vi "AIO-DAQ-Panel.vi"(7 "Set(F)":bool, 8 "error in (no error)":errorcluster, 10 "First Time(F)":bool, 11 "object in":refnum<class>) -> (0 "error out":errorcluster, 2 "Changed?":bool, 3 "object out":refnum<class>)   [LabVIEW 2021, in "DAQmx.lvlib" / "AIO-Configuration.lvclass"]
uses:
  AIO-Configuration.lvclass
  Dependencies/AIO-Channel.lvlibp/AIO-Configuration_class/tdef/Direction.ctl
  C:/Users/averna/Documents/LV Gym DEMO/Factory Pattern/Device Channels/Dependencies/AIO-Channel.lvlibp/Channels/AIO-Channel/AIO-Configuration_class/AIO-Configuration.lvclass
  tdef/Data.ctl
  AIO-Configuration.lvclass/AIO-Configuration.ctl
  <resource>/objmgr/daqmx.rc
  DAQmx.lvlib
  C:/Users/averna/Documents/LV Gym DEMO/Factory Pattern/Device Channels/Dependencies/AIO-Channel.lvlibp/AIO-Configuration_class/AIO-Configuration.lvclass
  C:/Users/averna/Documents/LV Gym DEMO/Factory Pattern/Device Channels/Dependencies/Channel.lvlibp/Channel/Configuration_class/Configuration.lvclass
  C:/Users/averna/Documents/LV Gym DEMO/Factory Pattern/Device Channels/DAQmx/AIO-Configuration_class/AIO-Configuration.lvclass
  Dependencies/AIO-Channel.lvlibp/AIO-Configuration_class/AIO-Configuration.lvclass
panel:
  in  "Units":string
  in  "Scale":string(combo)
  in  "input terminal configuration":i32(ring)=-1 items=["Default"=-1, "RSE"=10083, "NRSE"=10078, "Differential"=10106, "Pseudodifferential"=12529]
  in  "minimum value":dbl=-5.0 format="%0.2f"
  in  "maximum value":dbl=5.0 format="%0.2f"
  in  "Direction":T1
  in  "Line":string(combo)
  in  "Device":string(combo)
  out "Not Saved?":bool
  in  "Save":bool
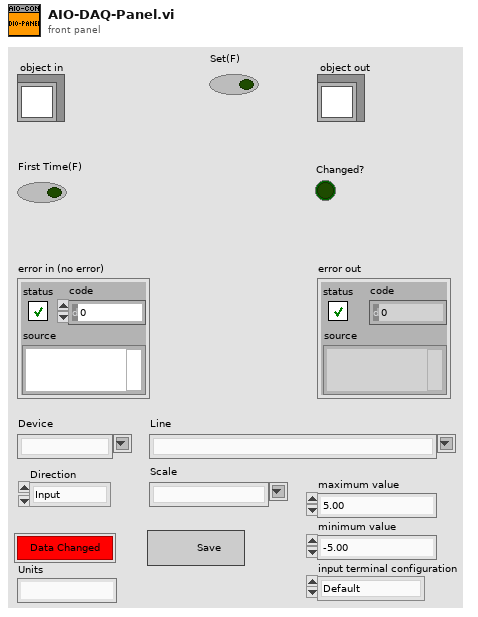
[diagram p1: front panel]
types:
  T1 = typedef "AIO-Channel.lvlibp/AIO-Configuration.lvclass/Direction.ctl" = enum16{"Input", "Output"}
  T2 = typedef "DAQmx.lvlib/AIO-Configuration.lvclass/Data.ctl" = cluster{"DAQ_Line":string, "maximum value":dbl, "minimum value":dbl, "input terminal configuration":i32, "custom scale name":string}
  T3 = cluster{"DAQ_Line":bool, "maximum value":bool, "minimum value":bool, "input terminal configuration":bool, "custom scale name":bool}
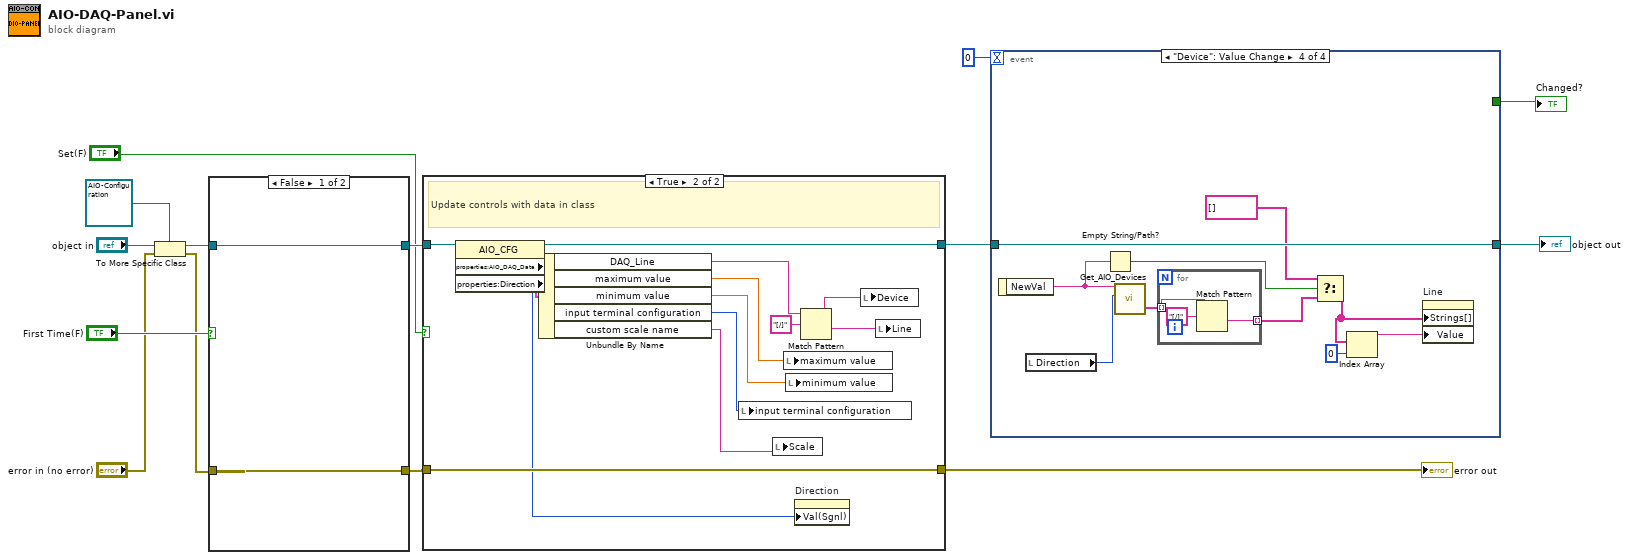
[diagram p0: block diagram]
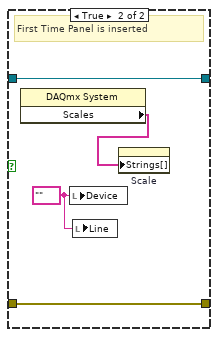
[diagram p2: hidden frame]
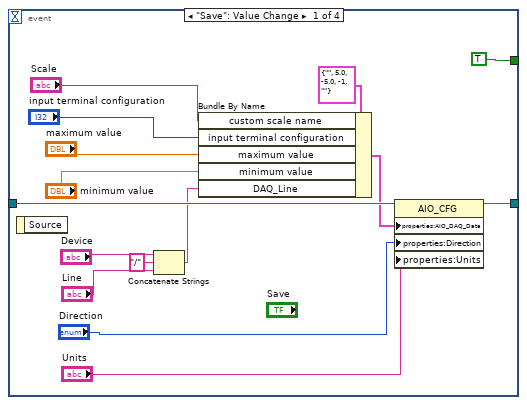
[diagram p3: hidden frame]
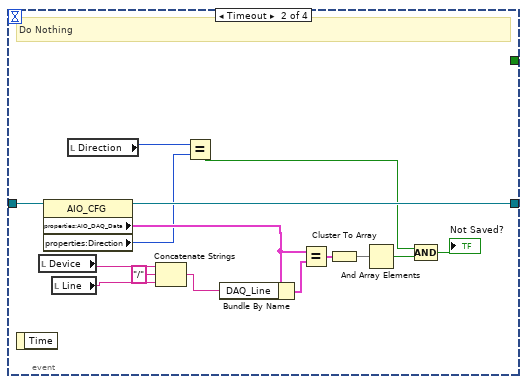
[diagram p4: hidden frame]
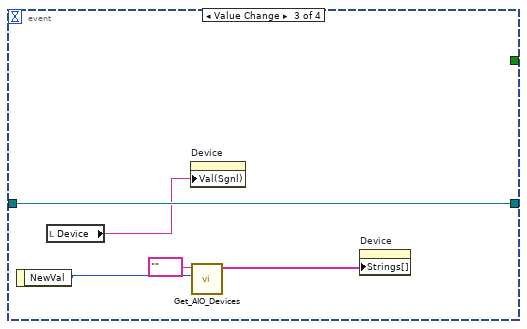
[diagram p5: hidden frame]
diagram:
  n1 = To More Specific Class(target class=refnum<class "AIO-Configuration.lvclass"> refnum ("Template-Channels.lvlib:Template_CFG"), reference="object in", error in="error in (no error)") -> (specific class reference=w8:refnum<class "AIO-Configuration.lvclass">, error out=w6:errorcluster)
  n2 = case shown="False" "First Time(F)" {
    tunnel: [w16 w20] -> w12
    tunnel: w8 -> [w16 w20]
    tunnel: [w15 w19] -> w11
    tunnel: w6 -> [w15 w19]
    frame False {
    }
    frame True {
      w18 = "" ("Device")
      # "First Time Panel is inserted"
      n3 = property class="DAQmx System"() -> ("Scales"=w17:tag[])  [unwired: 2 in, 2 out]
      n4 = local write "Device"(w18) -> ()
      n5 = local write "Line"(w18) -> ()
      n6 = property on="Scale" class="CmbBox"("Strings[]"=w17) -> ()  [unwired: 2 in, 2 out]
    }
  }
  n7 = case shown="True" "Set(F)" {
    tunnel: [w22 w33] -> w3
    tunnel: w12 -> [w22 w35]
    tunnel: [w21 w34] -> w10
    tunnel: w11 -> [w21 w34]
    frame False {
    }
    frame True {
      # "Update controls with data in class"
      n8 = property class="AIO_CFG"(reference=w35) -> (reference out=w33:refnum<class "AIO-Configuration.lvclass">, "properties:AIO_DAQ_Data"=w32:T2, "properties:Direction"=w27:T1)  [unwired: 1 in, 1 out]
      n9 = Unbundle By Name(w32) -> ("DAQ_Line"=w31:string, "maximum value"=w25:dbl, "minimum value"=w24:dbl, "input terminal configuration"=w26:i32, "custom scale name"=w23:string)
      n10 = local write "input terminal configuration"(w26) -> ()
      n11 = local write "Scale"(w23) -> ()
      n12 = local write "maximum value"(w25) -> ()
      n13 = local write "minimum value"(w24) -> ()
      n14 = property on="Direction" class="Enum (strict)"("Val(Sgnl)"=w27) -> ()  [unwired: 2 in, 2 out]
      n15 = Match Pattern(string=w31, regular expression="[/]") -> (before substring=w29:string, after substring=w28:string)  [unwired: 1 in, 2 out]
      n16 = local write "Device"(w29) -> ()
      n17 = local write "Line"(w28) -> ()
    }
  }
  "error out" <- w10
  n18 = event shown="[3] \"Device\": Value Change" {
    selector: _ -> [_ _ _ _]
    dyn-events: _ -> [_ _ _ _]
    timeout: 0 -> [_ _ _ _]
    tunnel: [w50 w64 w70 w80] -> w4
    tunnel: w3 -> [w49 w65 w70 w80]
    tunnel: [TRUE ("Changed?") _ _ _] -> w1
    event "Save": Value Change {
      n19 = event-data() -> ()  [unwired: 1 in, 1 out]
      n20 = Concatenate Strings("Device", "/" ("string"), "Line") -> (w37:string)
      n21 = Bundle By Name(cluster=T2 {"DAQ_Line"="", "maximum value"=5.0, "minimum value"=-5.0, "input terminal configuration"=-1, "custom scale name"=""} ("AIO_DAQ_Data"), "custom scale name"="Scale", "input terminal configuration"="input terminal configuration", "maximum value"="maximum value", "minimum value"="minimum value", "DAQ_Line"=w37) -> (w42:T2)
      n22 = property class="AIO_CFG"(reference=w49, "properties:AIO_DAQ_Data"=w42, "properties:Direction"="Direction", "properties:Units"="Units") -> (reference out=w50:refnum<class "AIO-Configuration.lvclass">)  [unwired: 1 in, 1 out]
    }
    event Timeout {
      # "Do Nothing"
      n23 = event-data() -> ()  [unwired: 1 in, 1 out]
      n24 = local read "Device"() -> (w58:string)
      n25 = property class="AIO_CFG"(reference=w65) -> (reference out=w64:refnum<class "AIO-Configuration.lvclass">, "properties:AIO_DAQ_Data"=w60:T2, "properties:Direction"=w53:T1)  [unwired: 1 in, 1 out]
      n26 = local read "Line"() -> (w57:string)
      n27 = local read "Direction"() -> (w54:T1)
      n28 = Concatenate Strings(w58, "/" ("string"), w57) -> (w55:string)
      n29 = Equal?(x=w54, y=w53) -> (x = y?=w51:bool)
      n30 = Bundle By Name(cluster=w60, "DAQ_Line"=w55) -> (w59:T2)
      n31 = Equal?(x=w60, y=w59) -> (x = y?=w63:T3)
      n32 = Cluster To Array(cluster=w63) -> (array=w62:bool[])
      n33 = And Array Elements(Boolean array=w62) -> (logical AND=w61:bool)
      n34 = Compound Arithmetic op=AND(w51, w61) -> (→"Not Saved?":bool)
    }
    event Value Change {
      n35 = event-data() -> ("NewVal"=w69:T1)  [unwired: 1 in]
      n36 = local read "Device"() -> (w67:string)
      n37 = property on="Device" class="CmbBox"("Val(Sgnl)"=w67) -> ()  [unwired: 2 in, 2 out]
      n38 = call "Get_AIO_Devices.vi"("Direction"=w69, "Device"=tag "") -> ("Devices"=w68:tag[])  [unwired: 7 in, 2 out]
      n39 = property on="Device" class="CmbBox"("Strings[]"=w68) -> ()  [unwired: 2 in, 2 out]
    }
    event "Device": Value Change {
      n40 = event-data() -> ("NewVal"=w75:string)  [unwired: 1 in]
      n41 = local read "Direction"() -> (w76:T1)
      n42 = Empty String/Path?(string/path=w75) -> (empty?=w72:bool)
      n43 = call "Get_AIO_Devices.vi"("Direction"=w76, "Device"=w75) -> ("Lines"=w77:tag[])  [unwired: 7 in, 2 out]
      n44 = for {
        tunnel: [w82] -> w73 mode=indexing
        tunnel: w77 -> [w81] mode=indexing
        n45 = Match Pattern(string=w81, regular expression="[/]") -> (after substring=w82:string)  [unwired: 1 in, 3 out]
      }
      n46 = Select(t=string[] [], s=w72, f=w73) -> (s? t:f=w74:string[])
      n47 = Index Array(array=w74, index=0) -> (element=w79:string)
      n48 = property on="Line" class="CmbBox"("Strings[]"=w74, "Value"=w79) -> ()  [unwired: 2 in, 2 out]
    }
  }
  "object out" <- w4
  "Changed?" <- w1
